vi "Read Raw.vi"(8 "error in (no error)":errorcluster, 10 "Data In":u8[](array[numeric]), 11 "Raw Reader Reference":T1 {"refnum" format="%.0x"}) -> (0 "error out":errorcluster, 1 "Data Length":u32, 2 "Data Out":u8[](array[numeric]), 4 "Data Offset":u32)   [LabVIEW 2021, in "Iceoryx.lvlib"]
uses:
  Iceoryx.lvlib
  Refnum/Typedef/BB Raw Reader Refnum.ctl
  SubVIs/Convert Error Core.vi
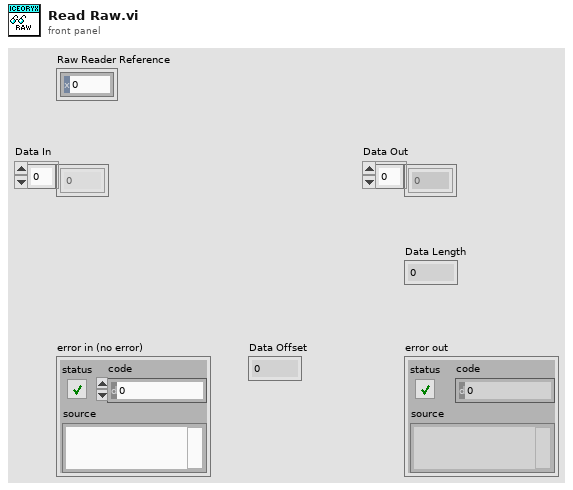
[diagram p1: front panel]
types:
  T1 = typedef "Iceoryx.lvlib/BB Raw Reader Refnum.ctl" = cluster{"refnum":u64, "BB Raw Reader":enum8{"bb_raw_reader"}}
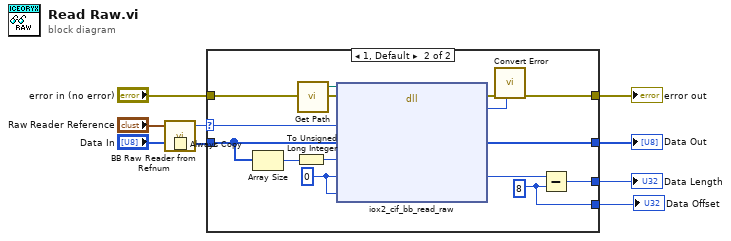
[diagram p0: block diagram]
diagram:
  n1 = call "BB Raw Reader from Refnum.vi"("BB Raw Reader Refnum"="Raw Reader Reference") -> ("BB Raw Reader U64"=w3:u64)  [unwired: 4 in]
  n2 = Always Copy(1:"Data In") -> (0:w1:u8[])
  n3 = case shown="1, Default" w3 {
    selector: w3 -> [_ w20]
    tunnel: "error in (no error)" -> [w11 w25]
    tunnel: w1 -> [w10 w19]
    tunnel: [w10 w15] -> w6
    tunnel: [w11 w21] -> w8
    tunnel: [_ w13] -> w5
    tunnel: [_ w12] -> w4
    frame 0 {
    }
    frame 1, Default {
      w12 = u32 8 ("Data Offset")
      w16 = u32 0 ("actual")
      n4 = Array Size(array=w19) -> (size(s)=w18:i32)
      n5 = To Unsigned Long Integer(number=w18) -> (unsigned 32bit integer=w17:u32)
      n6 = call "Get Path.vi"() -> ("libiox2_cif path"=w24:path)  [unwired: 4 in]
      n7 = dll-call lib="D:/dev/iceoryx2_lvwrapper/dist/iox2_cif.dll" fn="iox2_cif_bb_read_raw"(path in=w24, error in=w25, "reader"=w20, "bytes"=w19, "cap_bytes"=w17, "actual_bytes"=w16, "max_bytes"=w16) -> (error out=w23:errorcluster, "return type"=w22:i32, "bytes"=w15:u8[], "actual_bytes"=w14:u32)  [unwired: 4 in, 1 out]
      n8 = call "Convert Error.vi"("return type"=w22, "error in (no error)"=w23) -> ("error out"=w21:errorcluster)  [unwired: 9 in]
      n9 = Subtract(x=w14, y=w12) -> (x-y=w13:u32)
    }
  }
  "error out" <- w8
  "Data Out" <- w6
  "Data Length" <- w5
  "Data Offset" <- w4
